vi "Main.vi"() -> ()   [LabVIEW 2026]
uses:
  <vilib>/Instr/_visa.llb/VISA Configure Serial Port (Instr).vi
panel:
  out "SALIDA PWM":dbl(graph)
  in  "Modo":bool=TRUE
  in  "RESET":bool
  out "Maquina":T1(ring)
  in  "EMERGENCIA":bool
  in  "PWM":dbl min=0.0 max=100.0
  out "SP Vs ALTURA":cluster{dbl, dbl}(graph)
  out "PING PONG":dbl(slide) scale=0.0..50.0
  out "PID":enum16{"NO CONFIGURADO", "CONFIGURADO"}(ring)
  out "error out":errorcluster
  out "Enum":enum16{"DESCONECTADO", "CONECTADO"}(ring)
  out "ESTADO  SYS":enum16{"DETENIDO", "EJECUTANDO", "ERROR"}(ring)
  in  "PARADA":bool
  in  "INICIO":bool
  out "PID":string
  in  "SP":dbl=25.0 min=0.0 max=100.0
  in  "KD":dbl=0.07 min=0.0 max=65535.0
  in  "KI":dbl=0.14 min=0.0 max=65535.0
  in  "KP":dbl=3.9 min=0.0 max=65535.0
  in  "PID":bool
  out "SALIDA PID":dbl format="%.2g"
  out "ERROR":dbl format="%.2g"
  out "ALTURA":dbl format="%.2g"
  out "SP":dbl format="%.2f"
  out "array":string[][](array[string])
  out "Procesar":string
  in  "Stop Simulation":bool
  in  "Numeric":u32=115200
  in  "VISA resource name":refnum<visa-resource-name>="COM12"
  out "Iteracion":i32
  # "Sistema Levitador Neumático"
  # "Planta"
  # "Grafico en Tiempo Real"
  # "COMUNICACIÓN"
  # "ESTADO DEL SISTEMA"
  # "Estado :"
  # "Puerto :"
  # "Comunicación :"
  # "Baud :"
  # "Estado PID :"
  # "CONFIGURACIÓN PID"
  # "VARIABLES EN TIEMPO REAL"
  # "KP :"
  # "KI  :"
  # "KD :"
  # "AUTO"
  # "MANUAL"
  # "SP :"
  # "PWM :"
  # "Mensaje a Procesar :"
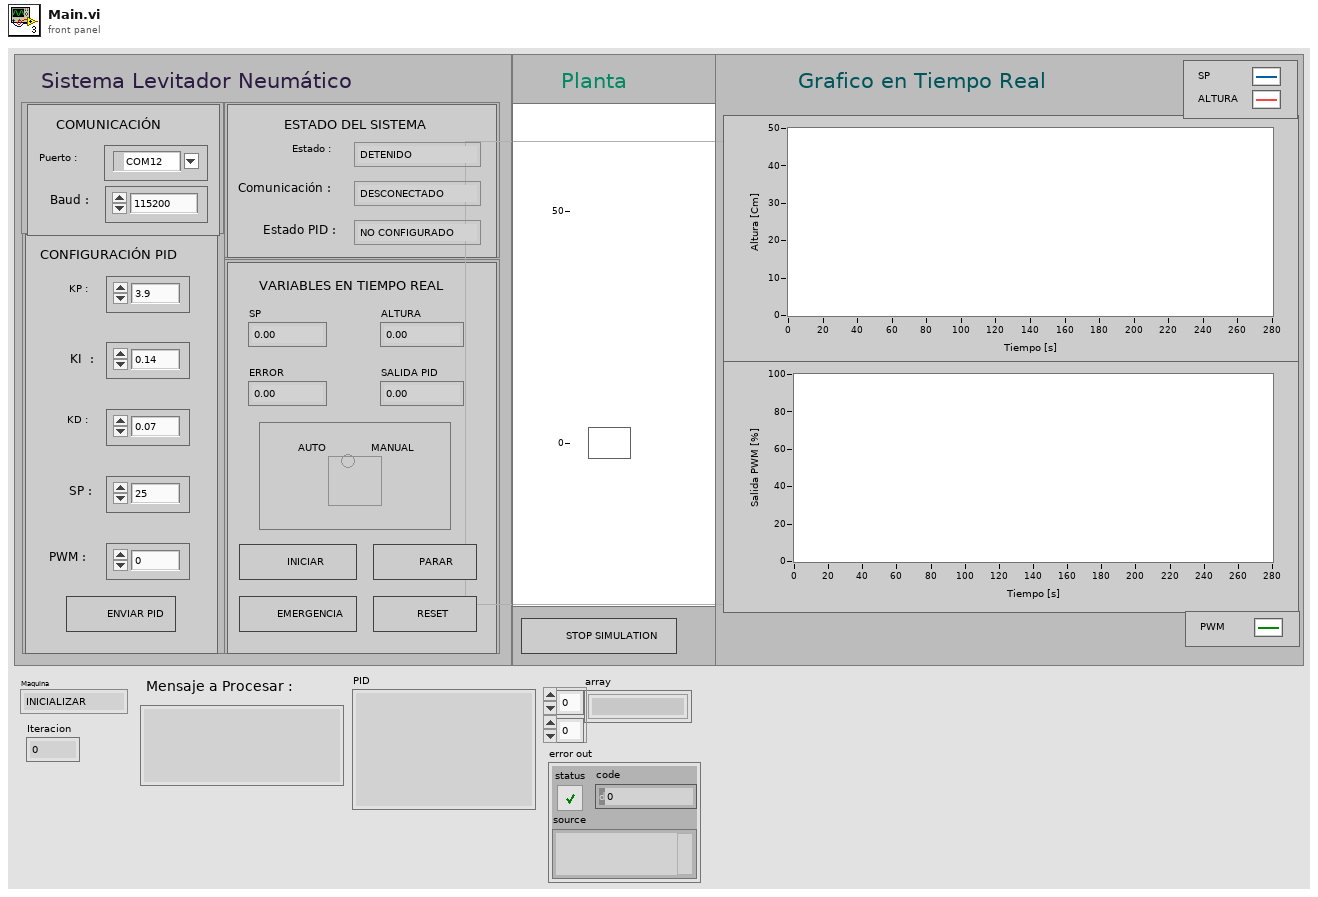
[diagram p1: front panel]
types:
  T1 = enum16{"INICIALIZAR", "ESPERA", "ENVIAR_MODO", "ENVIAR_SP", "ENVIAR_PID", "RECIBIR", "PROCESAR", "ENVIAR_RESET", "ENVIAR_RUN", "ENVIAR_STOP", "ENVIAR_EMERGENCIA_ON", "ENVIAR_EMERGENCIA_OFF", "ERROR", "CERRAR"}
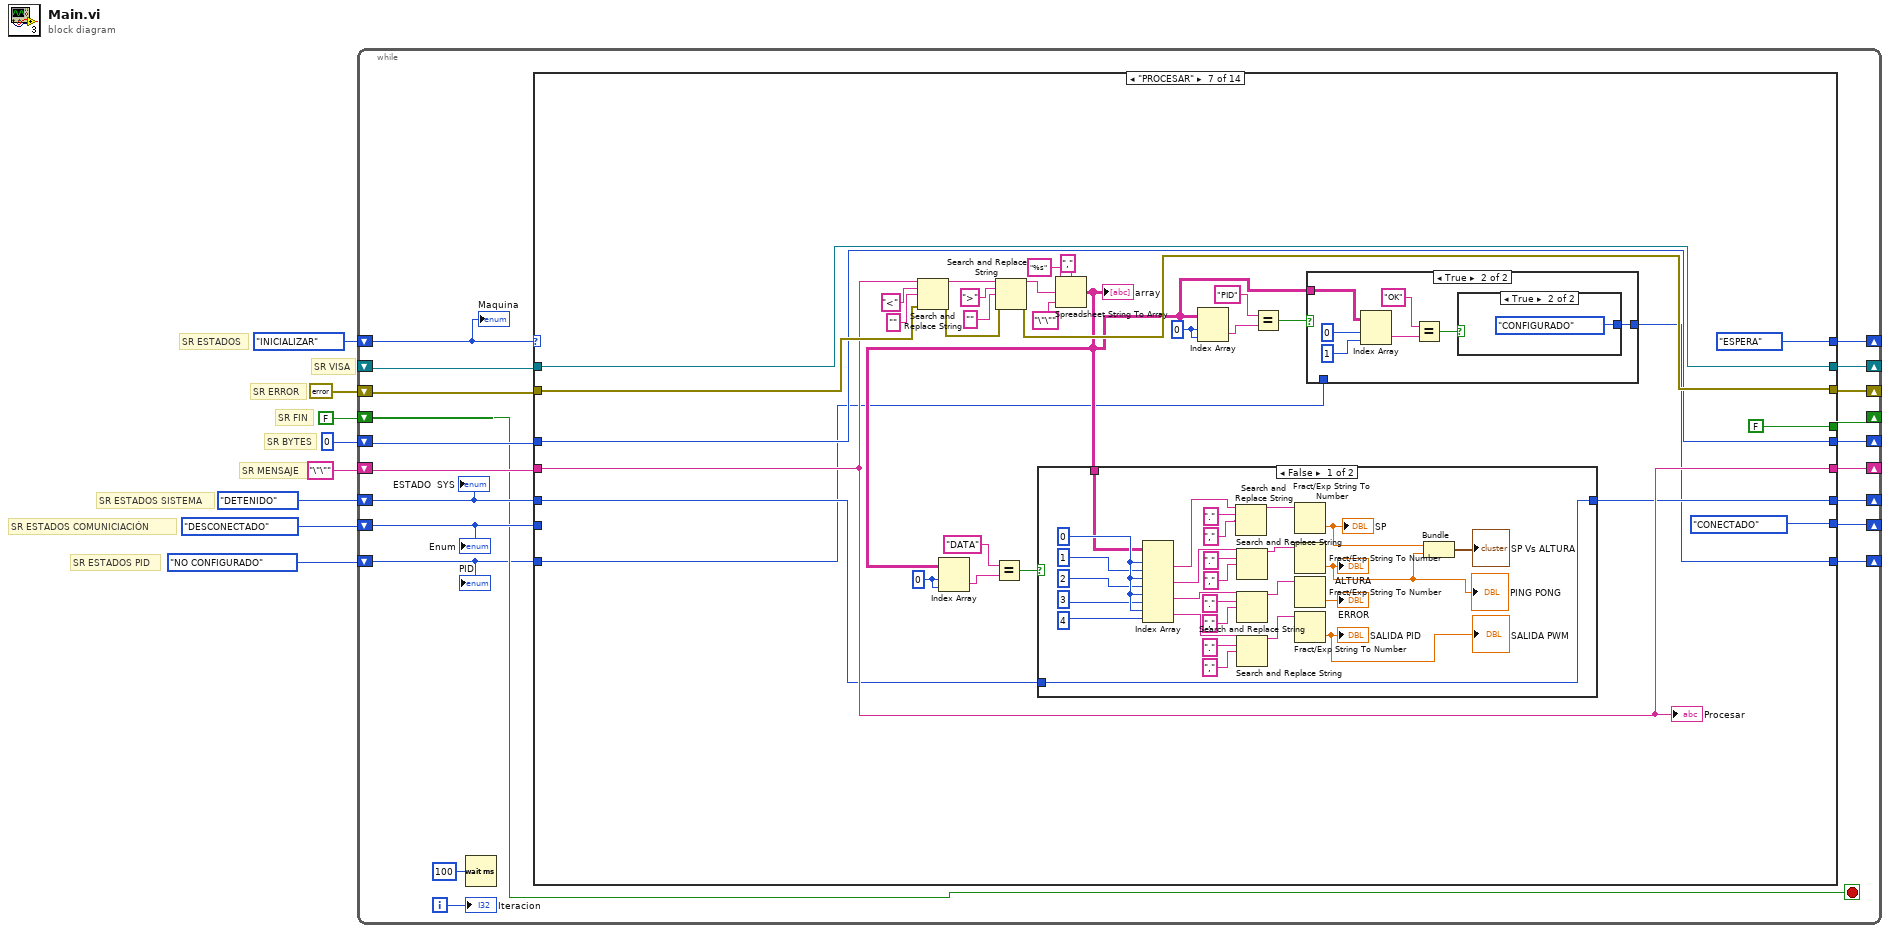
[diagram p0: block diagram]
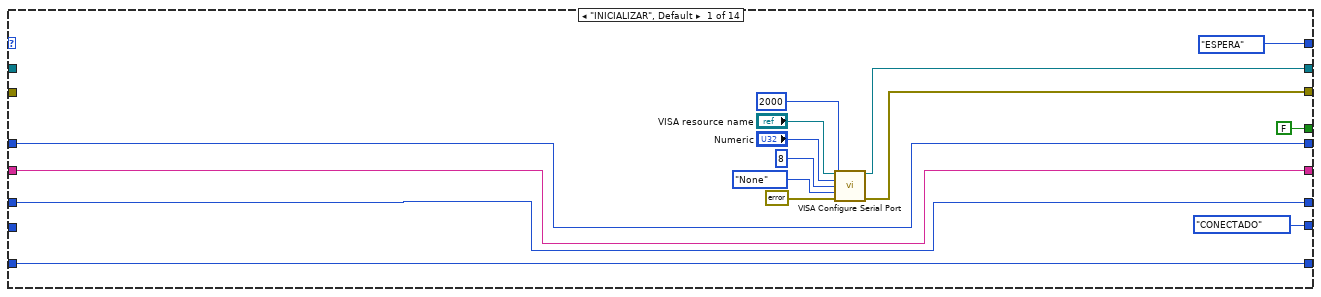
[diagram p2: hidden frame]
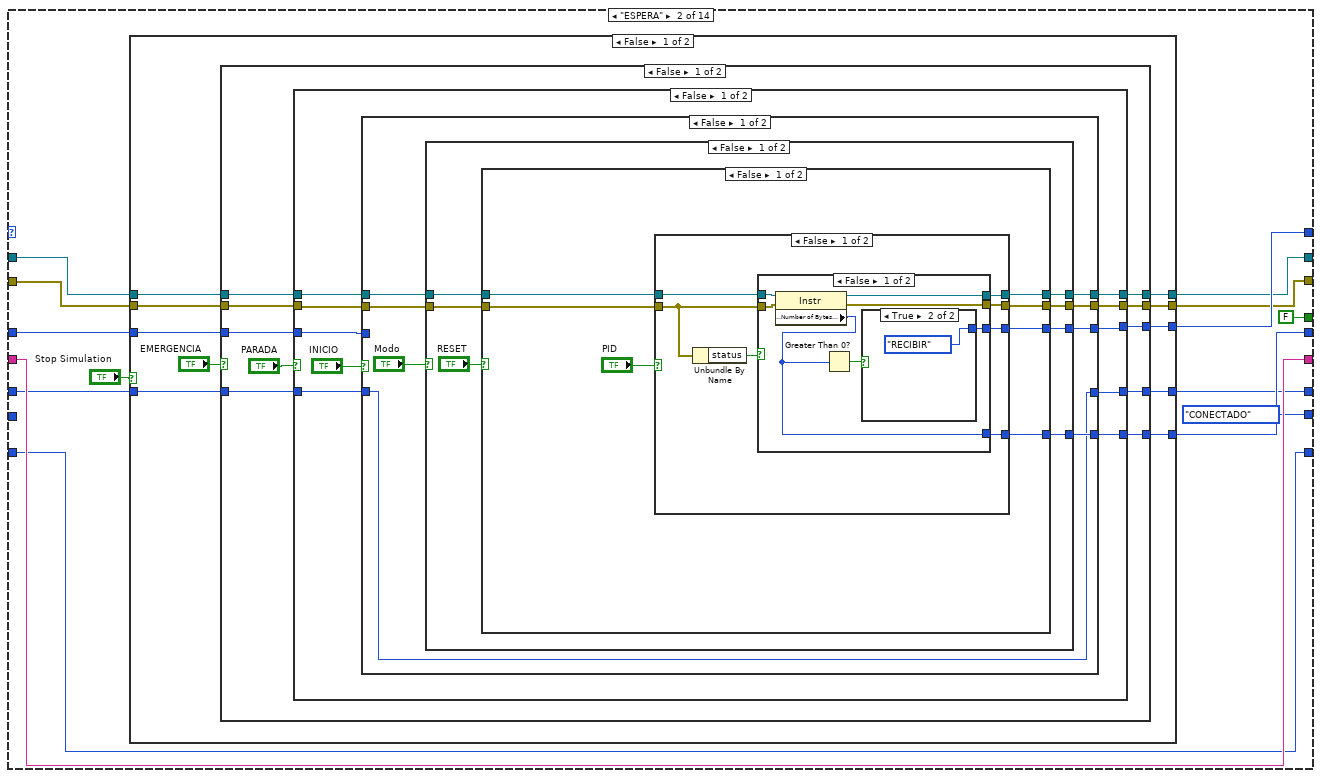
[diagram p3: hidden frame]
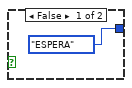
[diagram p4: hidden frame]
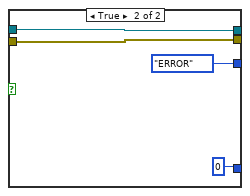
[diagram p5: hidden frame]
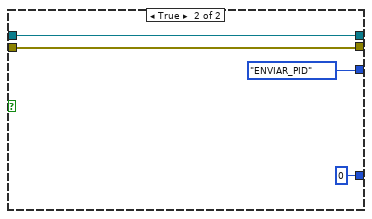
[diagram p6: hidden frame]
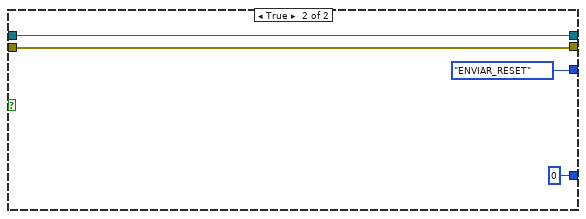
[diagram p7: hidden frame]
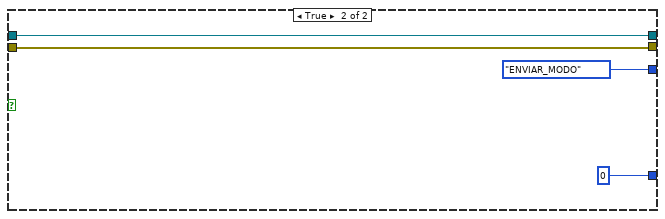
[diagram p8: hidden frame]
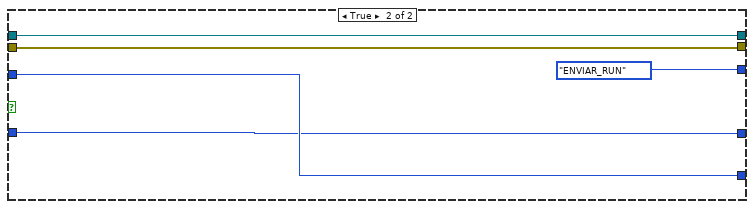
[diagram p9: hidden frame]
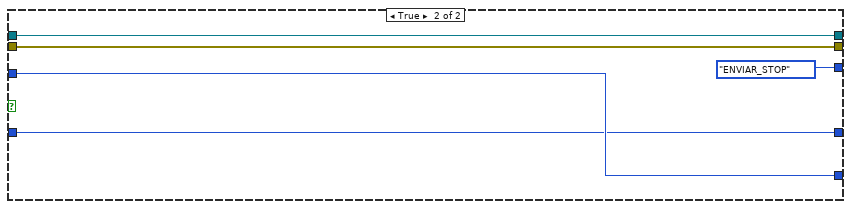
[diagram p10: hidden frame]
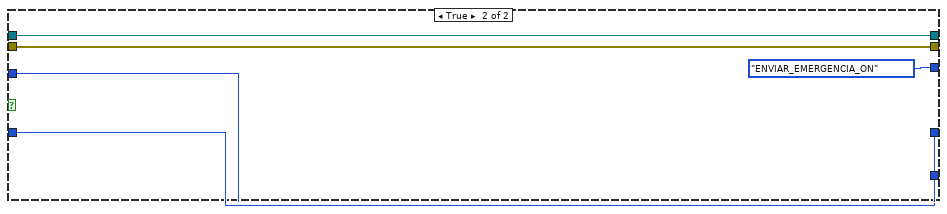
[diagram p11: hidden frame]
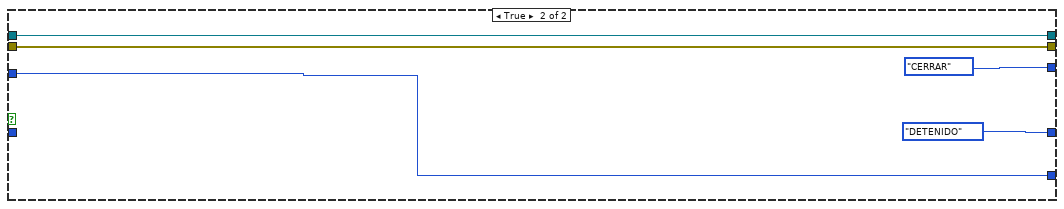
[diagram p12: hidden frame]
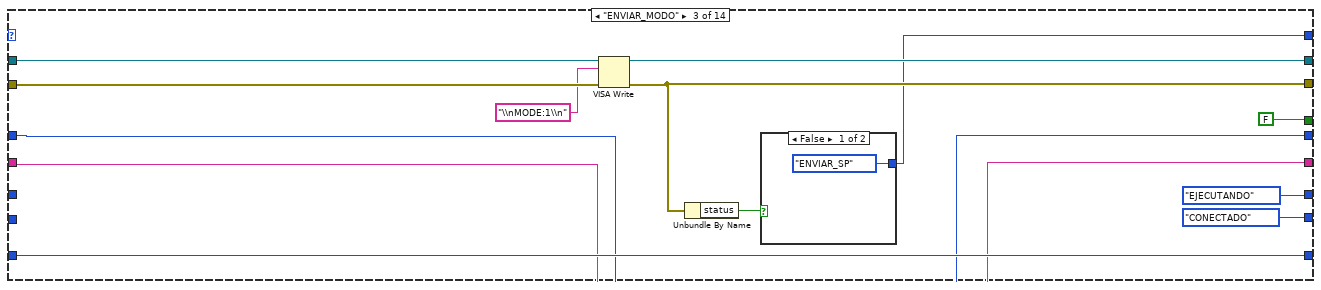
[diagram p13: hidden frame]
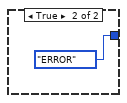
[diagram p14: hidden frame]
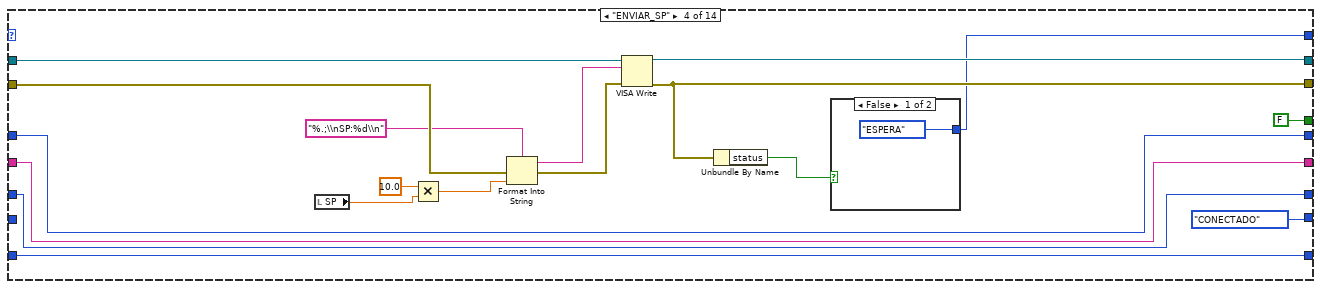
[diagram p15: hidden frame]
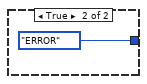
[diagram p16: hidden frame]
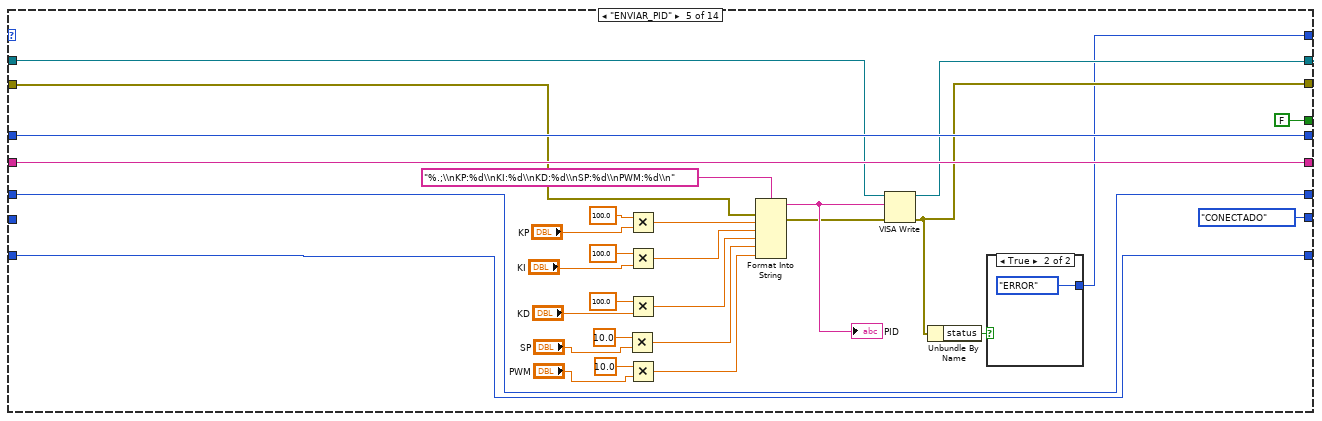
[diagram p17: hidden frame]
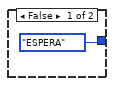
[diagram p18: hidden frame]
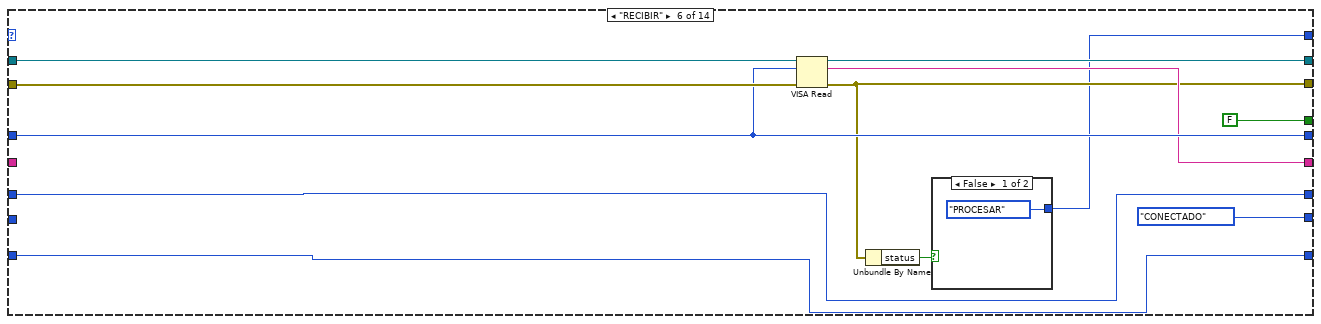
[diagram p19: hidden frame]
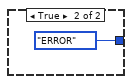
[diagram p20: hidden frame]
diagram:
  # "SR ESTADOS PID"
  # "SR ESTADOS COMUNICIACIÓN"
  # "SR ESTADOS SISTEMA"
  # "SR MENSAJE"
  # "SR BYTES"
  # "SR FIN"
  # "SR ERROR"
  # "SR ESTADOS"
  # "SR VISA"
  n1 = while {
    shift-right: [w26] -> _
    shift-left: _ -> [w24]
    shift-right: [w25] -> _
    shift-left: errorcluster {"status"=FALSE, "code"=0, "source"=""} ("error out") -> [w23]
    shift-right: [w22] -> _
    shift-left: FALSE -> [w13]
    shift-right: [w21] -> _
    shift-left: u32 0 ("Bytes at Port") -> [w20]
    shift-right: [w19] -> _
    shift-left: "\"\"" -> [w18]
    shift-right: [w14] -> _
    shift-left: enum16{"DETENIDO", "EJECUTANDO", "ERROR"}."DETENIDO" -> [w16]
    shift-right: [w15] -> _
    shift-left: enum16{"DESCONECTADO", "CONECTADO"}."DESCONECTADO" -> [w17]
    shift-right: [w11] -> _
    shift-left: enum16{"NO CONFIGURADO", "CONFIGURADO"}."NO CONFIGURADO" -> [w12]
    shift-right: [w9] -> _
    shift-left: T1."INICIALIZAR" -> [w10]
    i -> [w28]
    stop <- w13 stop-if-true
    n2 = Wait (ms)(milliseconds to wait=u32 100) -> ()  [unwired: 1 out]
    n3 = case shown="\"PROCESAR\"" w10 {
      tunnel: [T1."ESPERA" w57 w167 w183 w215 w232 T1."ESPERA" w326 w345 w358 w374 w390 T1."CERRAR" T1."CERRAR"] -> w9
      tunnel: [w37 w54 w168 w192 w220 w237 w273 w329 w347 w359 w371 w392 w407 w410] -> w26
      tunnel: [w36 w53 w169 w191 w217 w234 w264 w321 w346 w360 w370 w391 w402 w411] -> w25
      tunnel: w24 -> [_ w55 w171 w194 w221 w239 w273 w331 w349 w364 w376 w394 w407 w410]
      tunnel: w23 -> [_ w49 w170 w190 w223 w238 w265 w330 w348 w363 w375 w393 w402 w412]
      tunnel: [FALSE FALSE FALSE FALSE FALSE FALSE FALSE FALSE FALSE FALSE FALSE FALSE FALSE TRUE] -> w22
      tunnel: [w34 w52 w162 w177 w225 w236 w260 w325 w342 w361 w372 w385 w405 w416] -> w21
      tunnel: w20 -> [w34 w51 w162 w177 w225 w236 w260 w325 w342 w361 w372 w385 w405 w416]
      tunnel: [w33 w50 w163 w178 w224 w235 w257 w324 w343 w362 w369 w384 w404 w415] -> w19
      tunnel: w18 -> [w33 w50 w163 w178 w224 _ w257 w324 w343 w362 w369 w384 w404 w415]
      tunnel: w16 -> [w31 w46 _ w180 w213 w230 w251 w323 _ _ _ _ w401 _]
      tunnel: w17 -> [_ _ _ _ _ _ _ _ _ _ _ _ _ _]
      tunnel: [enum16{"DESCONECTADO", "CONECTADO"}."CONECTADO" enum16{"DESCONECTADO", "CONECTADO"}."CONECTADO" enum16{"DESCONECTADO", "CONECTADO"}."CONECTADO" enum16{"DESCONECTADO", "CONECTADO"}."CONECTADO" enum16{"DESCONECTADO", "CONECTADO"}."CONECTADO" enum16{"DESCONECTADO", "CONECTADO"}."CONECTADO" enum16{"DESCONECTADO", "CONECTADO"}."CONECTADO" enum16{"DESCONECTADO", "CONECTADO"}."CONECTADO" enum16{"DESCONECTADO", "CONECTADO"}."CONECTADO" enum16{"DESCONECTADO", "CONECTADO"}."CONECTADO" enum16{"DESCONECTADO", "CONECTADO"}."CONECTADO" enum16{"DESCONECTADO", "CONECTADO"}."CONECTADO" enum16{"DESCONECTADO", "CONECTADO"}."CONECTADO" enum16{"DESCONECTADO", "CONECTADO"}."DESCONECTADO"] -> w15
      tunnel: [w31 w47 enum16{"DETENIDO", "EJECUTANDO", "ERROR"}."EJECUTANDO" w180 w213 w230 w252 w323 enum16{"DETENIDO", "EJECUTANDO", "ERROR"}."EJECUTANDO" enum16{"DETENIDO", "EJECUTANDO", "ERROR"}."DETENIDO" enum16{"DETENIDO", "EJECUTANDO", "ERROR"}."EJECUTANDO" enum16{"DETENIDO", "EJECUTANDO", "ERROR"}."EJECUTANDO" w401 enum16{"DETENIDO", "EJECUTANDO", "ERROR"}."DETENIDO"] -> w14
      tunnel: w12 -> [w30 w44 w164 w181 w212 w229 w244 w322 w339 w354 w373 w386 w400 w409]
      tunnel: [w30 w44 w164 w181 w212 w229 w245 w322 w339 w354 w373 w386 w400 w409] -> w11
      frame "INICIALIZAR", Default {
        n4 = call-poly "VISA Configure Serial Port"("VISA resource name"="VISA resource name", "timeout (10sec)"=u32 2000, "baud rate (9600)"="Numeric", "data bits (8)"=u16 8, "parity (0:none)"=enum16{"None", "Odd", "Even", "Mark", "Space"}."None", "error in (no error)"=errorcluster {"status"=FALSE, "code"=0, "source"=""}) -> ("VISA resource name out"=w37:refnum<visa-resource-name>, "error out"=w36:errorcluster)  [unwired: 8 in]
      }
      frame "ESPERA" {
        n5 = case shown="False" "Stop Simulation" {
          tunnel: [w67 T1."CERRAR"] -> w57
          tunnel: w55 -> [w66 w159]
          tunnel: [w65 w159] -> w54
          tunnel: [w64 w158] -> w53
          tunnel: [w63 w161] -> w52
          tunnel: w51 -> [w62 w161]
          tunnel: w49 -> [w61 w158]
          tunnel: [w60 enum16{"DETENIDO", "EJECUTANDO", "ERROR"}."DETENIDO"] -> w47
          tunnel: w46 -> [w59 _]
          frame False {
            n6 = case shown="False" "EMERGENCIA" {
              tunnel: [w77 T1."ENVIAR_EMERGENCIA_ON"] -> w67
              tunnel: w66 -> [w69 w154]
              tunnel: [w76 w154] -> w65
              tunnel: [w75 w153] -> w64
              tunnel: [w74 w156] -> w63
              tunnel: w62 -> [w73 w156]
              tunnel: w61 -> [w68 w153]
              tunnel: [w71 w155] -> w60
              tunnel: w59 -> [w70 w155]
              frame False {
                n7 = case shown="False" "PARADA" {
                  tunnel: [w87 T1."ENVIAR_STOP"] -> w77
                  tunnel: w69 -> [w86 w151]
                  tunnel: w68 -> [w85 w150]
                  tunnel: [w84 w151] -> w76
                  tunnel: [w83 w150] -> w75
                  tunnel: [w82 w149] -> w74
                  tunnel: w73 -> [w80 w149]
                  tunnel: [w79 w148] -> w71
                  tunnel: w70 -> [w78 w148]
                  frame False {
                    n8 = case shown="False" "INICIO" {
                      tunnel: [w95 T1."ENVIAR_RUN"] -> w87
                      tunnel: w86 -> [w94 w146]
                      tunnel: w85 -> [w93 w145]
                      tunnel: [w92 w146] -> w84
                      tunnel: [w91 w145] -> w83
                      tunnel: [w90 w144] -> w82
                      tunnel: w80 -> [_ w144]
                      tunnel: [w89 w143] -> w79
                      tunnel: w78 -> [w89 w143]
                      frame False {
                        n9 = case shown="False" "Modo" {
                          tunnel: [w102 T1."ENVIAR_MODO"] -> w95
                          tunnel: w94 -> [w101 w141]
                          tunnel: w93 -> [w100 w140]
                          tunnel: [w99 w141] -> w92
                          tunnel: [w98 w140] -> w91
                          tunnel: [w97 u32 0 ("Bytes at Port")] -> w90
                          frame False {
                            n10 = case shown="False" "RESET" {
                              tunnel: [w109 T1."ENVIAR_RESET"] -> w102
                              tunnel: w101 -> [w107 w137]
                              tunnel: w100 -> [w106 w136]
                              tunnel: [w105 w137] -> w99
                              tunnel: [w104 w136] -> w98
                              tunnel: [w103 u32 0 ("Bytes at Port")] -> w97
                              frame False {
                                n11 = case shown="False" "PID" {
                                tunnel: [w116 T1."ENVIAR_PID"] -> w109
                                tunnel: w107 -> [w115 w132]
                                tunnel: w106 -> [w111 w131]
                                tunnel: [w114 w132] -> w105
                                tunnel: [w113 w131] -> w104
                                tunnel: [w112 u32 0 ("Bytes at Port")] -> w103
                                frame False {
                                n12 = Unbundle By Name(w111) -> ("status"=w110:bool)
                                n13 = case shown="False" w110 {
                                tunnel: [w123 T1."ERROR"] -> w116
                                tunnel: w115 -> [w122 w129]
                                tunnel: w111 -> [w121 w128]
                                tunnel: [w120 w129] -> w114
                                tunnel: [w119 w128] -> w113
                                tunnel: [w117 u32 0 ("Bytes at Port")] -> w112
                                frame False {
                                n14 = property class="Instr"(reference=w122, error in=w121) -> (reference out=w120:refnum<visa-resource-name>, error out=w119:errorcluster, "Serial Settings:Number of Bytes at Serial Port"=w117:u32)
                                n15 = Greater Than 0?(x=w117) -> (x > 0?=w118:bool)
                                n16 = case shown="True" w118 {
                                tunnel: [T1."ESPERA" T1."RECIBIR"] -> w123
                                frame False {
                                }
                                frame True {
                                }
                                }
                                }
                                frame True {
                                }
                                }
                                }
                                frame True {
                                }
                                }
                              }
                              frame True {
                              }
                            }
                          }
                          frame True {
                          }
                        }
                      }
                      frame True {
                      }
                    }
                  }
                  frame True {
                  }
                }
              }
              frame True {
              }
            }
          }
          frame True {
          }
        }
      }
      frame "ENVIAR_MODO" {
        n17 = VISA Write(VISA resource name=w171, write buffer="\\nMODE:1\\n", error in (no error)=w170) -> (VISA resource name out=w168:refnum<visa-resource-name>, error out=w169:errorcluster)  [unwired: 1 out]
        n18 = Unbundle By Name(w169) -> ("status"=w165:bool)
        n19 = case shown="False" w165 {
          tunnel: [T1."ENVIAR_SP" T1."ERROR"] -> w167
          frame False {
          }
          frame True {
          }
        }
      }
      frame "ENVIAR_SP" {
        n20 = local read "SP"() -> (w186:dbl)
        n21 = Multiply(x=10.0, y=w186) -> (x*y=w188:dbl)
        n22 = Format Into String(format string="%.;\\nSP:%d\\n", error in=w190, w188) -> (resulting string=w184:string, error out=w185:errorcluster)  [unwired: 1 in]
        n23 = VISA Write(VISA resource name=w194, write buffer=w184, error in (no error)=w185) -> (VISA resource name out=w192:refnum<visa-resource-name>, error out=w191:errorcluster)  [unwired: 1 out]
        n24 = Unbundle By Name(w191) -> ("status"=w193:bool)
        n25 = case shown="False" w193 {
          tunnel: [T1."ESPERA" T1."ERROR"] -> w183
          frame False {
          }
          frame True {
          }
        }
      }
      frame "ENVIAR_PID" {
        n26 = Multiply(x=10.0, y="SP") -> (x*y=w200:dbl)
        n27 = Multiply(x=100.0, y="KP") -> (x*y=w203:dbl)
        n28 = Multiply(x=100.0, y="KI") -> (x*y=w207:dbl)
        n29 = Multiply(x=100.0, y="KD") -> (x*y=w211:dbl)
        n30 = Multiply(x=10.0, y="PWM") -> (x*y=w197:dbl)
        n31 = Format Into String(format string="%.;\\nKP:%d\\nKI:%d\\nKD:%d\\nSP:%d\\nPWM:%d\\n", error in=w223, w203, w207, w211, w200, w197) -> (resulting string=w222:string, error out=w218:errorcluster)  [unwired: 1 in]
        "PID" <- w222
        n32 = VISA Write(VISA resource name=w221, write buffer=w222, error in (no error)=w218) -> (VISA resource name out=w220:refnum<visa-resource-name>, error out=w217:errorcluster)  [unwired: 1 out]
        n33 = Unbundle By Name(w217) -> ("status"=w216:bool)
        n34 = case shown="True" w216 {
          tunnel: [T1."ESPERA" T1."ERROR"] -> w215
          frame False {
          }
          frame True {
          }
        }
      }
      frame "RECIBIR" {
        n35 = VISA Read(VISA resource name=w239, byte count=w236, error in (no error)=w238) -> (VISA resource name out=w237:refnum<visa-resource-name>, read buffer=w235:string, error out=w234:errorcluster)  [unwired: 1 out]
        n36 = Unbundle By Name(w234) -> ("status"=w233:bool)
        n37 = case shown="False" w233 {
          tunnel: [T1."PROCESAR" T1."ERROR"] -> w232
          frame False {
          }
          frame True {
          }
        }
      }
      frame "PROCESAR" {
        w250 = 0 ("index (row)")
        w256 = 0 ("index (row)")
        n38 = Search and Replace String(input string=w257, search string="<", replace string="" ("replace string (\"\")"), error in=w265) -> (result string=w269:string, error out=w268:errorcluster)  [unwired: 4 in, 2 out]
        n39 = Search and Replace String(input string=w269, search string=">", replace string="" ("replace string (\"\")"), error in=w268) -> (result string=w262:string, error out=w264:errorcluster)  [unwired: 4 in, 2 out]
        n40 = Spreadsheet String To Array(delimiter (Tab)=",", format string="%s", spreadsheet string=w262, array type (2D Dbl)="\"\"") -> (array=w246:string[][])
        "array" <- w246
        n41 = Index Array(array=w246, index (row)=w256, index (col)=w256) -> (element=w255:string)
        n42 = Equal?(x="DATA", y=w255) -> (x = y?=w253:bool)
        n43 = case shown="False" w253 {
          tunnel: w246 -> [w287 w318]
          tunnel: [w286 w312] -> w252
          tunnel: w251 -> [w286 _]
          frame False {
            w311 = 0 ("index (row)")
            n44 = Index Array(array=w287, index (row) #1=w311, index (col) #1=1 ("index"), index (row) #2=w311, index (col) #2=2 ("index"), index (row) #3=w311, index (col) #3=3 ("index"), index (row) #4=w311, index (col) #4=4 ("index")) -> (element #1=w305:string, element #2=w296:string, element #3=w295:string, element #4=w294:string)
            n45 = Search and Replace String(input string=w305, search string=".", replace string="," ("replace string (\"\")")) -> (result string=w303:string)  [unwired: 5 in, 3 out]
            n46 = Search and Replace String(input string=w296, search string=".", replace string="," ("replace string (\"\")")) -> (result string=w292:string)  [unwired: 5 in, 3 out]
            n47 = Search and Replace String(input string=w295, search string=".", replace string="," ("replace string (\"\")")) -> (result string=w291:string)  [unwired: 5 in, 3 out]
            n48 = Search and Replace String(input string=w294, search string=".", replace string="," ("replace string (\"\")")) -> (result string=w290:string)  [unwired: 5 in, 3 out]
            n49 = Fract/Exp String To Number(string=w303) -> (number=w289:dbl)  [unwired: 3 in, 1 out]
            "SP" <- w289
            n50 = Fract/Exp String To Number(string=w292) -> (number=w285:dbl)  [unwired: 3 in, 1 out]
            "ALTURA" <- w285
            "PING PONG" <- w285
            n51 = Fract/Exp String To Number(string=w291) -> (number=→"ERROR":dbl)  [unwired: 3 in, 1 out]
            n52 = Fract/Exp String To Number(string=w290) -> (number=→"SALIDA PID" →"SALIDA PWM":dbl)  [unwired: 3 in, 1 out]
            n53 = Bundle(w289, w285) -> (→"SP Vs ALTURA":cluster{dbl, dbl})  [unwired: 1 in]
          }
          frame True {
            n54 = Index Array(array=w318, index (row)=0, index (col)=1 ("disabled index (col)")) -> (element=w315:string)
            n55 = Equal?(x="RUN", y=w315) -> (x = y?=w313:bool)
            n56 = case shown="True" w313 {
              tunnel: [enum16{"DETENIDO", "EJECUTANDO", "ERROR"}."DETENIDO" enum16{"DETENIDO", "EJECUTANDO", "ERROR"}."EJECUTANDO"] -> w312
              frame False {
              }
              frame True {
              }
            }
          }
        }
        n57 = Index Array(array=w246, index (row)=w250, index (col)=w250) -> (element=w249:string)
        n58 = Equal?(x="PID", y=w249) -> (x = y?=w247:bool)
        n59 = case shown="True" w247 {
          tunnel: w246 -> [_ w277]
          tunnel: [w274 w275] -> w245
          tunnel: w244 -> [w274 _]
          frame False {
          }
          frame True {
            n60 = Index Array(array=w277, index (row)=0, index (col)=1 ("disabled index (col)")) -> (element=w279:string)
            n61 = Equal?(x="OK", y=w279) -> (x = y?=w276:bool)
            n62 = case shown="True" w276 {
              tunnel: [enum16{"NO CONFIGURADO", "CONFIGURADO"}."NO CONFIGURADO" enum16{"NO CONFIGURADO", "CONFIGURADO"}."CONFIGURADO"] -> w275
              frame False {
              }
              frame True {
              }
            }
          }
        }
        "Procesar" <- w257
      }
      frame "ENVIAR_RESET" {
        w332 = 0.0 ("input 1")
        n63 = Format Into String(format string="%.;\\nKP:%d\\nKI:%d\\nKD:%d\\nSP:%d\\nPWM:%d\\n", error in=w330, w332, w332, w332, w332, w332) -> (resulting string=w336:string, error out=w334:errorcluster)  [unwired: 1 in]
        n64 = VISA Write(VISA resource name=w331, write buffer=w336, error in (no error)=w334) -> (VISA resource name out=w329:refnum<visa-resource-name>, error out=w321:errorcluster)  [unwired: 1 out]
        n65 = Unbundle By Name(w321) -> ("status"=w333:bool)
        n66 = case shown="False" w333 {
          tunnel: [T1."ESPERA" T1."ERROR"] -> w326
          frame False {
          }
          frame True {
          }
        }
      }
      frame "ENVIAR_RUN" {
        n67 = VISA Write(VISA resource name=w349, write buffer="\\nEN:1\\n", error in (no error)=w348) -> (VISA resource name out=w347:refnum<visa-resource-name>, error out=w346:errorcluster)  [unwired: 1 out]
        n68 = Unbundle By Name(w346) -> ("status"=w351:bool)
        n69 = case shown="True" w351 {
          tunnel: [T1."ESPERA" T1."ERROR"] -> w345
          frame False {
          }
          frame True {
          }
        }
      }
      frame "ENVIAR_STOP" {
        n70 = VISA Write(VISA resource name=w364, write buffer="\\nEN:0\\n", error in (no error)=w363) -> (VISA resource name out=w359:refnum<visa-resource-name>, error out=w360:errorcluster)  [unwired: 1 out]
        n71 = Unbundle By Name(w360) -> ("status"=w366:bool)
        n72 = case shown="True" w366 {
          tunnel: [T1."ESPERA" T1."ERROR"] -> w358
          frame False {
          }
          frame True {
          }
        }
      }
      frame "ENVIAR_EMERGENCIA_ON" {
        n73 = VISA Write(VISA resource name=w376, write buffer="\\nEMG:1\\n", error in (no error)=w375) -> (VISA resource name out=w371:refnum<visa-resource-name>, error out=w370:errorcluster)  [unwired: 1 out]
        n74 = Unbundle By Name(w370) -> ("status"=w381:bool)
        n75 = case shown="False" w381 {
          tunnel: [T1."ESPERA" T1."ERROR"] -> w374
          frame False {
          }
          frame True {
          }
        }
      }
      frame "ENVIAR_EMERGENCIA_OFF" {
        n76 = VISA Write(VISA resource name=w394, write buffer="\\nEMG:0\\n", error in (no error)=w393) -> (VISA resource name out=w392:refnum<visa-resource-name>, error out=w391:errorcluster)  [unwired: 1 out]
        n77 = Unbundle By Name(w391) -> ("status"=w396:bool)
        n78 = case shown="False" w396 {
          tunnel: [T1."ESPERA" T1."ERROR"] -> w390
          frame False {
          }
          frame True {
          }
        }
      }
      frame "ERROR" {
        "error out" <- w402
      }
      frame "CERRAR" {
        n79 = VISA Close(VISA resource name=w410, error in (no error)=w412) -> (error out=w411:errorcluster)
      }
    }
    "Iteracion" <- w28
    "ESTADO  SYS" <- w16
    "Enum" <- w17
    "PID" <- w12
    "Maquina" <- w10
  }
